vi "Update RPC Client Method Constants.vi"(5 "Library":refnum<vi>, 6 "RPC Method Parameters":T1, 8 "error in (no error)":errorcluster, 11 "VI in":refnum<vi>) -> (0 "error out":errorcluster, 3 "VI out":refnum<vi>)   [LabVIEW 2019, in "gRPC Template Creation Utility.lvlib"]
uses:
  gRPC Template Creation Utility.lvlib
  TypeDefs/RPC Method Parameters.ctl
  <vilib>/Utility/traverseref.llb/TRef TravTarget.ctl
  Oneof API/OneOf Constants/OneOfConstantsEnum.ctl
  0eaa7444-8baf-4465-b530-593cae42fb70.vi
  <vilib>/Comparison/Equal/Equal Functor/Equal Functor.lvclass
  <vilib>/Utility/traverseref.llb/VI Scripting - Traverse.lvlib
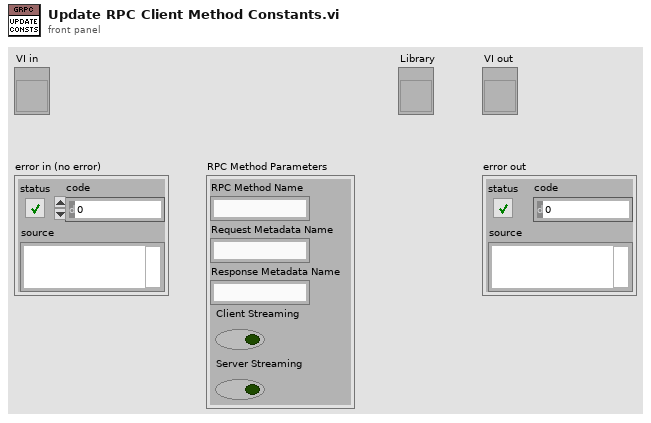
[diagram p1: front panel]
types:
  T1 = typedef "gRPC Template Creation Utility.lvlib/RPC Method Parameters.ctl" = cluster{"RPC Method Name":string, "Request Metadata Name":string, "Response Metadata Name":string, "Client Streaming":bool, "Server Streaming":bool}
  T2 = typedef "TRef TravTarget.ctl" = enum16{"FP", "BD", "Other"}
  T3 = typedef "gRPC Template Creation Utility.lvlib/OneOfConstantsEnum.ctl" = enum16{"FlatToRichVIPrefix", "RichToFlatVIPrefix", "FlatTypeDefSuffix"}
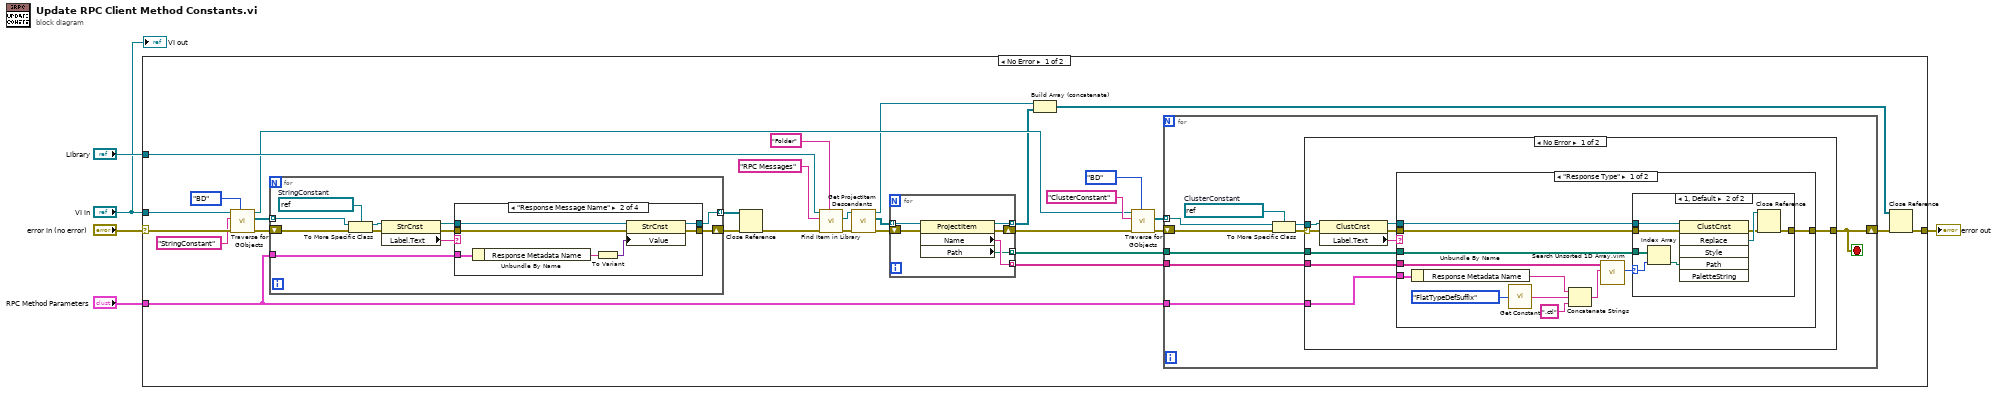
[diagram p0: block diagram]
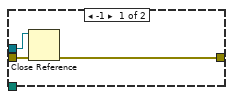
[diagram p2: hidden frame]
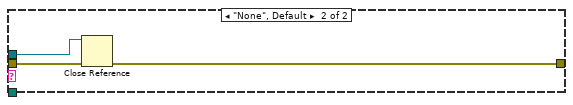
[diagram p3: hidden frame]
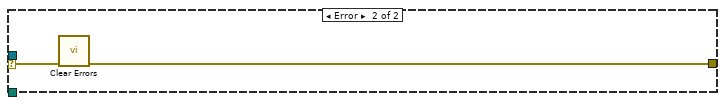
[diagram p4: hidden frame]
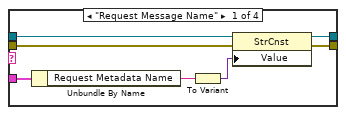
[diagram p5: hidden frame]
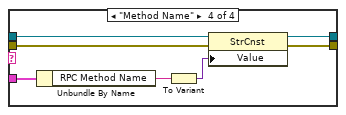
[diagram p7: hidden frame]
diagram:
  n1 = case shown="No Error" "error in (no error)" {
    selector: "error in (no error)" -> [w35 w122]
    tunnel: [w6 w122] -> w5
    tunnel: "VI in" -> [w34 _]
    tunnel: "Library" -> [w33 _]
    tunnel: "RPC Method Parameters" -> [w32 _]
    frame No Error {
      n2 = call <vilib>:"Traverse for GObjects.vi"("Traverse Target"=TRef_TravTarget."BD", "error in (no error)"=w35, "Class Name"="StringConstant", "VI Refnum"=w34) -> ("error out"=w29:errorcluster, "References"=w25:refnum<vi>[], "dup VI Refnum"=w10:refnum<vi>)  [unwired: 4 in, 1 out]
      n3 = for {
        tunnel: w25 -> [w97] mode=indexing
        shift-right: [w89] -> w26
        shift-left: w29 -> [w96]
        tunnel: w32 -> [w92]
        tunnel: [w88] -> w24 mode=indexing
        w98 = refnum<vi> refnum  # StringConstant
        n4 = To More Specific Class(target class=w98, reference=w97, error in=w96) -> (specific class reference=w95:refnum<vi>, error out=w94:errorcluster)
        n5 = property class="StrCnst"(reference=w95, error in=w94) -> (reference out=w91:refnum<vi>, error out=w90:errorcluster, "Label.Text"=w93:string)
        n6 = case shown="\"Response Message Name\"" w93 {
          tunnel: w92 -> [w100 w110 _ w121]
          tunnel: w91 -> [w102 w108 w113 w120]
          tunnel: w90 -> [w103 w109 w114 w117]
          tunnel: [w101 w107 w114 w116] -> w89
          tunnel: [w99 w106 w113 w115] -> w88
          frame "Request Message Name" {
            n7 = Unbundle By Name(w100) -> ("Request Metadata Name"=w105:string)
            n8 = To Variant(anything=w105) -> (Variant=w104:variant)
            n9 = property class="StrCnst"(reference=w102, error in=w103, "Value"=w104) -> (reference out=w99:refnum<vi>, error out=w101:errorcluster)
          }
          frame "Response Message Name" {
            n10 = Unbundle By Name(w110) -> ("Response Metadata Name"=w112:string)
            n11 = To Variant(anything=w112) -> (Variant=w111:variant)
            n12 = property class="StrCnst"(reference=w108, error in=w109, "Value"=w111) -> (reference out=w106:refnum<vi>, error out=w107:errorcluster)
          }
          frame "None", Default {
          }
          frame "Method Name" {
            n13 = Unbundle By Name(w121) -> ("RPC Method Name"=w119:string)
            n14 = To Variant(anything=w119) -> (Variant=w118:variant)
            n15 = property class="StrCnst"(reference=w120, error in=w117, "Value"=w118) -> (reference out=w115:refnum<vi>, error out=w116:errorcluster)
          }
        }
      }
      n16 = Close Reference(reference=w24, error in (no error)=w26) -> (error out=w16:errorcluster)
      n17 = call "Find Item in Library.vi"("Item Type"="Folder", "error in (no error)"=w16, "Item Name"="RPC Messages", "Library item in"=w33) -> ("error out"=w20:errorcluster, "Project Item (Library Item)"=w19:refnum<vi>)  [unwired: 4 in, 2 out]
      n18 = call "Get ProjectItem Descendants.vi"("error in (no error)"=w20, "ProjectItem in"=w19) -> ("error out"=w15:errorcluster, "All Descendents"=w21:refnum<vi>[], "ProjectItem out"=w9:refnum<vi>)  [unwired: 7 in]
      n19 = for {
        tunnel: w21 -> [w41] mode=indexing
        tunnel: [w40] -> w12 mode=indexing
        tunnel: [w39] -> w8 mode=indexing
        shift-right: [w37] -> w14
        shift-left: w15 -> [w38]
        tunnel: [w36] -> w11 mode=indexing
        n20 = property class="ProjectItem"(reference=w41, error in=w38) -> (reference out=w39:refnum<vi>, error out=w37:errorcluster, "Name"=w40:string, "Path"=w36:path)
      }
      n21 = Build Array (concatenate)(w9, w8) -> (w7:refnum<vi>[])
      n22 = call <vilib>:"Traverse for GObjects.vi"("Traverse Target"=TRef_TravTarget."BD", "error in (no error)"=w14, "Class Name"="ClusterConstant", "VI Refnum"=w10) -> ("error out"=w23:errorcluster, "References"=w22:refnum<vi>[])  [unwired: 4 in, 2 out]
      n23 = for {
        tunnel: w22 -> [w43] mode=indexing
        shift-right: [w42] -> w13
        shift-left: w23 -> [w49]
        tunnel: w32 -> [w46]
        tunnel: w12 -> [w45]
        tunnel: w11 -> [w44]
        stop <- w42 stop-if-true
        w50 = refnum<vi> refnum  # ClusterConstant
        n24 = To More Specific Class(target class=w50, reference=w43, error in=w49) -> (specific class reference=w48:refnum<vi>, error out=w47:errorcluster)
        n25 = case shown="No Error" w47 {
          selector: w47 -> [w58 w87]
          tunnel: w48 -> [w59 _]
          tunnel: [w54 w86] -> w42
          tunnel: w46 -> [w53 _]
          tunnel: w45 -> [w52 _]
          tunnel: w44 -> [w51 _]
          frame No Error {
            n26 = property class="ClustCnst"(reference=w59, error in=w58) -> (reference out=w56:refnum<vi>, error out=w55:errorcluster, "Label.Text"=w57:string)
            n27 = case shown="\"Response Type\"" w57 {
              tunnel: w56 -> [w65 w85]
              tunnel: w55 -> [w64 w84]
              tunnel: [w63 w83] -> w54
              tunnel: w53 -> [w71 _]
              tunnel: w52 -> [w69 _]
              tunnel: w51 -> [w67 _]
              frame "Response Type" {
                n28 = Unbundle By Name(w71) -> ("Response Metadata Name"=w62:string)
                n29 = call "Get Constant.vi"("Selection"=OneOfConstantsEnum."FlatTypeDefSuffix") -> ("String"=w60:string)
                n30 = Concatenate Strings(w62, w60, ".ctl" ("string")) -> (w68:string)
                n31 = call "Search Unsorted 1D Array.vim"("element"=w68, "unsorted 1D array"=w69) -> ("index of element"=w66:i32)  [unwired: 9 in]
                n32 = case shown="1, Default" w66 {
                  selector: w66 -> [_ w81]
                  tunnel: w67 -> [_ w82]
                  tunnel: w65 -> [w74 w80]
                  tunnel: w64 -> [w73 w79]
                  tunnel: [w72 w75] -> w63
                  frame -1 {
                    n33 = Close Reference(reference=w74, error in (no error)=w73) -> (error out=w72:errorcluster)
                  }
                  frame 1, Default {
                    n34 = Index Array(array=w82, index=w81) -> (element=w78:path)
                    n35 = invoke class="ClustCnst" method="Replace"(reference=w80, error in=w79, "Path"=w78) -> (error out=w76:errorcluster, "Replace"=w77:refnum<vi>)  [unwired: 3 in, 4 out]
                    n36 = Close Reference(reference=w77, error in (no error)=w76) -> (error out=w75:errorcluster)
                  }
                }
              }
              frame "None", Default {
                n37 = Close Reference(reference=w85, error in (no error)=w84) -> (error out=w83:errorcluster)
              }
            }
          }
          frame Error {
            n38 = call <vilib>:"Clear Errors.vi"("error in (no error)"=w87) -> ("error out"=w86:errorcluster)  [unwired: 5 in, 1 out]
          }
        }
      }
      n39 = Close Reference(reference=w7, error in (no error)=w13) -> (error out=w6:errorcluster)
    }
    frame Error {
    }
  }
  "error out" <- w5
  "VI out" <- "VI in"
